vi "from_string.vi"(7 "optional file path (to include in parse error message)":path, 8 "error in (no error)":errorcluster, 10 "toml":string) -> (0 "error out":errorcluster, 3 "toml out":refnum<class "toml.lvclass">)   [LabVIEW 2020, in "toml.lvclass"]
uses:
  toml.lvclass
  toml.lvclass/toml.ctl
  Doc/Doc.lvclass
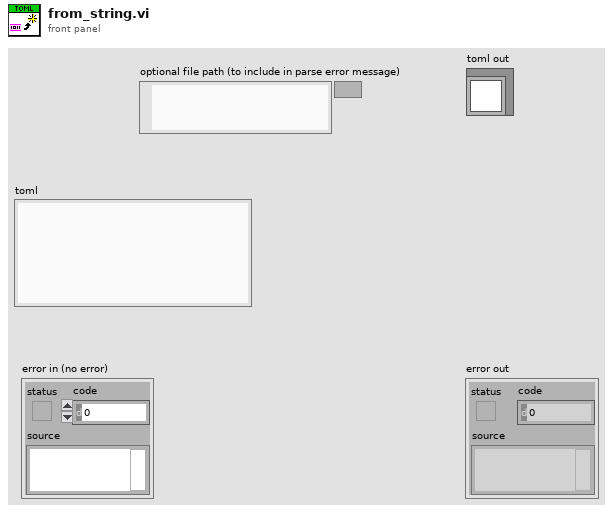
[diagram p1: front panel]
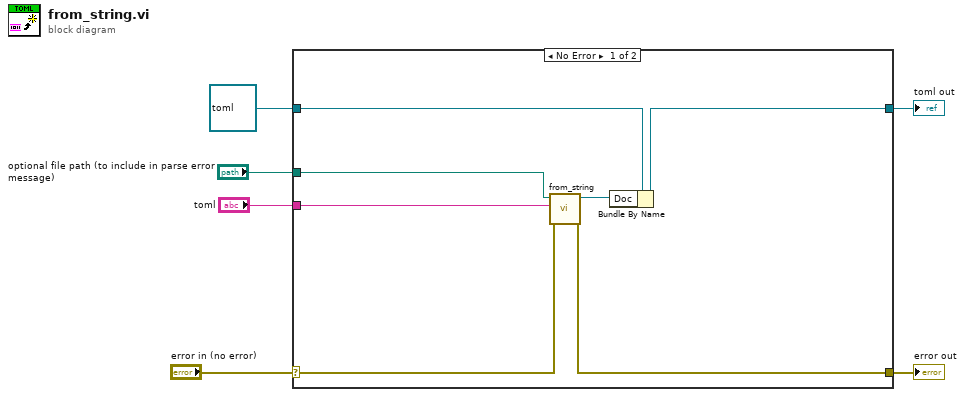
[diagram p0: block diagram]
diagram:
  n1 = case shown="No Error" "error in (no error)" {
    selector: "error in (no error)" -> [w9 w15]
    tunnel: [w8 w15] -> w5
    tunnel: [w11 w14] -> w3
    tunnel: refnum<class "toml.lvclass"> refnum ("toml in") -> [w13 w14]
    tunnel: "toml" -> [w12 _]
    tunnel: "optional file path (to include in parse error message)" -> [w7 _]
    frame No Error {
      n2 = call "from_string.vi"("error in (no error)"=w9, "toml"=w12, "file path (to include in error message)"=w7) -> ("error out"=w8:errorcluster, "Doc out"=w10:refnum<class "Doc.lvclass">)  [unwired: 7 in]
      n3 = Bundle By Name(cluster=w13, "Doc"=w10) -> (w11:refnum<class "toml.lvclass">)
    }
    frame Error {
    }
  }
  "error out" <- w5
  "toml out" <- w3
